vi "FPGA Main.vi"() -> ()   [LabVIEW 2016]
doc: "This FPGA Main VI contains a control loop running in parallel with an RT watchdog loop.\n- The Control Loop performs control calculations on four input channels in parallel, and outputs the results to four output channels.\n- The RT Watchdog Loop checks for a periodic 'pet' from the RT Main VI to ensure communications between RT and FPGA are maintained."
uses:
  <vilib>/LabVIEW Targets/FPGA/cRIO/shared/nicrio_ModuleControls/nicrio_cRIO-9239_DataRatesRing.ctl
  <vilib>/rvi/Emulation/niFpgaGetClockAttributes.vi
  <vilib>/rvi/Emulation/niFpgaSctlEmulationGetInTimedLoop.vi
  <vilib>/rvi/Emulation/niFpgaEmulationReportErrorSimple.vi
  <vilib>/rvi/Emulation/niFpgaProcessEmulError.vi
  <vilib>/rvi/eio/common/nirviEmuTemplatePropertySet_errors.vi
  <vilib>/rvi/eio/common/nirviEmuTemplateMethod_errors.vi
  <vilib>/rvi/interface/RandomDataEmulation/niFpgaRandomDataHandleErrors.vi
  <vilib>/rvi/Emulation/niFpgaCriticalErrorInLSC.vi
  <vilib>/eio/EIOPropertyNode/EIOPropertyNode.xnode
  <vilib>/eio/EIONode/EIONode.xnode
  <vilib>/rvi/DataTransferAndStorage/Container/XNode/niFpgaContainer.xnode
  <vilib>/rvi/interface/RandomDataEmulation/nirviRandomDataFpgaReadWriteTemplate.vi
  <vilib>/rvi/FXPMathLib/FxpMul/XNode/nifxpmath_Multiplier.xnode
  <vilib>/rvi/eio/common/nirviEmuTemplatePropertyGet_errors.vi
  <vilib>/rvi/eio/common/nirviEmuTemplatePropertyGet_noerrors.vi
  <vilib>/rvi/eio/common/nirviEmuTemplatePropertySet_noerrors.vi
  <vilib>/rvi/FXPMathLib/sim/FxpSim.dll
panel:
  in  "Stop":bool
  out "AI FIFO Full":bool
  out "AI AO Error":errorcluster
  out "AO FIFO Empty":bool
  in  "Loop Rate(uSec)":u32 caption="Loop Rate (uSec)"
  in  "Stop":bool
  in  "Amplitude":fxp<+/-,20,5>=10.0
  in  "Frequency (periods/tick)":fxp<+,32,0>=1.2499978765845299e-05
  in  "Data Rate":T1=1 items=["50.000 kS/s (NI 9239)"=1, "25.000 kS/s (NI 9239)"=2, "16.667 kS/s (NI 9239)"=3, "12.500 kS/s (NI 9239)"=4, "10.000 kS/s (NI 9239)"=5, "8.333 kS/s (NI 9239)"=6, "7.143 kS/s (NI 9239)"=7, "6.250 kS/s (NI 9239)"=8, "5.556 kS/s (NI 9239)"=9, "5.000 kS/s (NI 9239)"=10, "4.545 kS/s (NI 9239)"=11, "4.167 kS/s (NI 9239)"=12, "3.846 kS/s (NI 9239)"=13, "3.571 kS/s (NI 9239)"=14, "3.333 kS/s (NI 9239)"=15, "3.125 kS/s (NI 9239)"=16, "2.941 kS/s (NI 9239)"=17, "2.778 kS/s (NI 9239)"=18, "2.632 kS/s (NI 9239)"=19, "2.500 kS/s (NI 9239)"=20, "2.381 kS/s (NI 9239)"=21, "2.273 kS/s (NI 9239)"=22, "2.174 kS/s (NI 9239)"=23, "2.083 kS/s (NI 9239)"=24, "2.000 kS/s (NI 9239)"=25, "1.923 kS/s (NI 9239)"=26, "1.852 kS/s (NI 9239)"=27, "1.786 kS/s (NI 9239)"=28, "1.724 kS/s (NI 9239)"=29, "1.667 kS/s (NI 9239)"=30, "1.613 kS/s (NI 9239)"=31]
  out "FPGA Error":errorcluster
  out "Finished":bool
  in  "Stop":bool
  out "Module Underflow":bool
  out "DMA FIFO Full":bool
  out "Different Channel Count":bool
  out "Actual Loop Period (ticks)":u32
  out "First Read":bool
  in  "Number of Channels":i32=16
  in  "Channel Scale Array":fxp<+,24,12>[](array[numeric])=[0.0, 0.0, 0.0, 0.0, 0.0, 0.0, 0.0, 0.0, 0.0, 0.0, 0.0, 0.0, 0.0, 0.0, 0.0, 0.0]
  # "Essa VI é a interface direta entre o software (LabVIEW) e a FPGA.\nQualquer alteração mínima nela deve ser compilada, o que leva em torno de 20 minutos,  para poder ser executada."
  # "Reception Settings"
  # "Monitoring Values"
  # "Transmission"
  # "Supervision Analog"
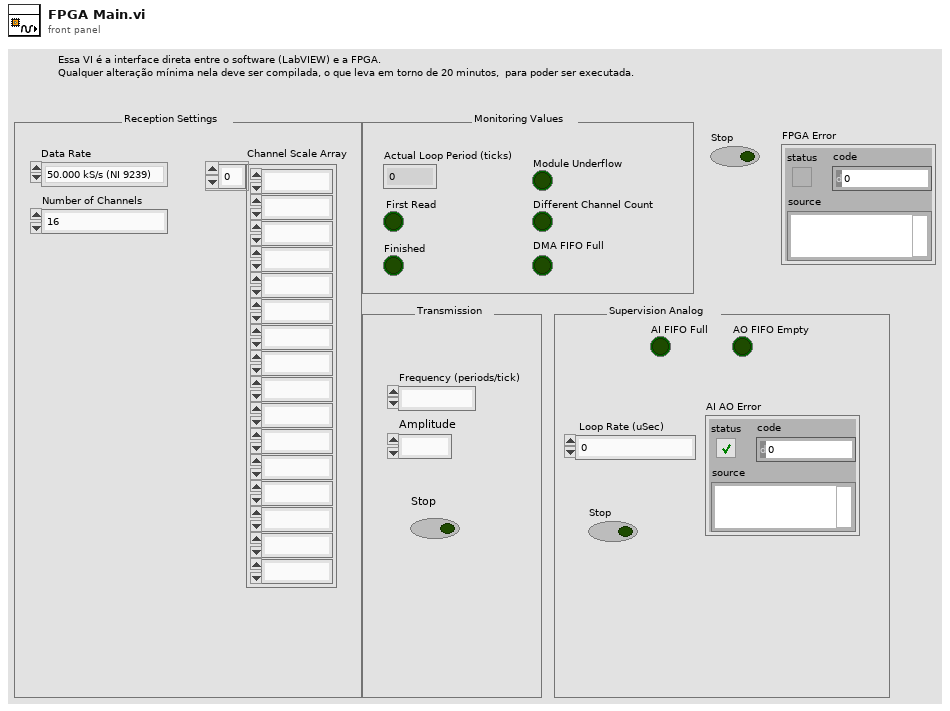
[diagram p1: front panel]
types:
  T1 = typedef "nicrio_cRIO-9239_DataRatesRing.ctl" = u8
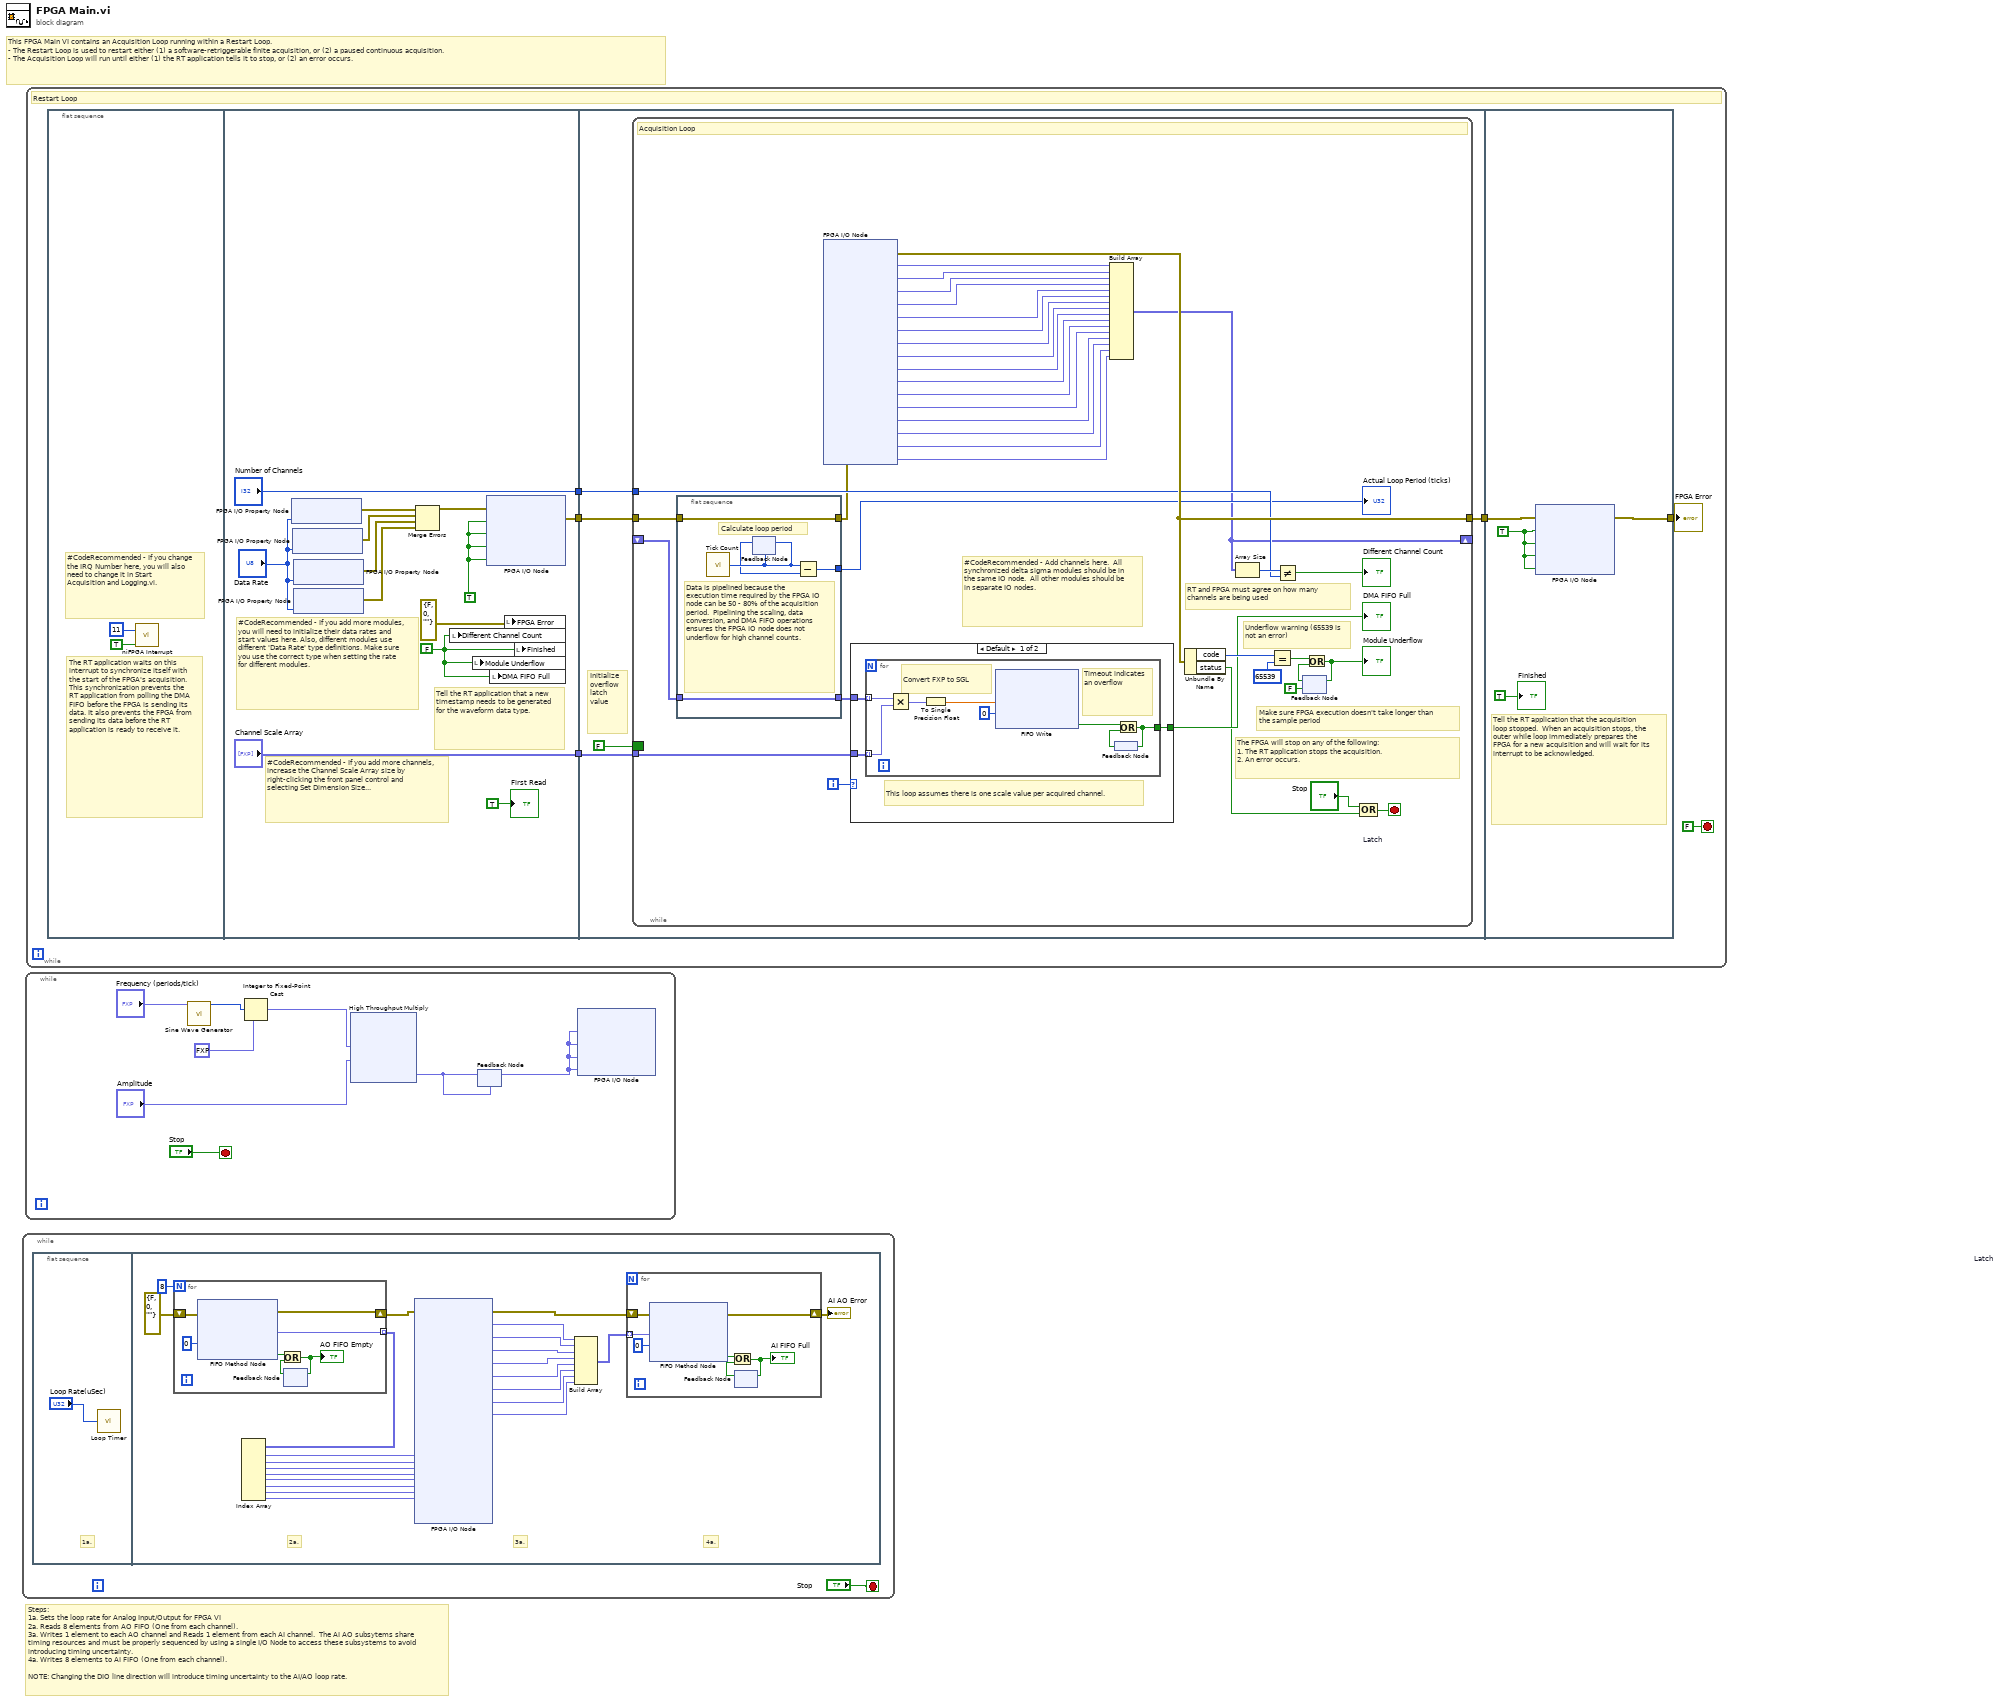
[diagram p0: block diagram]
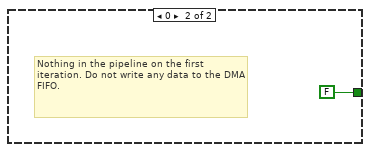
[diagram p2: hidden frame]
diagram:
  # "Steps:\n1a. Sets the loop rate for Analog Input/Output for FPGA VI\n2a. Reads 8 elements from AO FIFO (One from each channel).\n3a. Writes 1 element to each AO channel and Reads 1 element from each AI channel.  The AI AO subsytems share timing resources and must be properly sequenced by using a single I/O Node to access these subsystems to avoid introducing timing uncertainty.\n4a. Writes 8 elements to AI FIFO (One from each channel).\n\nNOTE: Changing the DIO line direction will introduce timing uncertainty to the AI/AO loop rate."
  # "This FPGA Main VI contains an Acquisition Loop running within a Restart Loop.\n- The Restart Loop is used to restart either (1) a software-retriggerable finite acquisition, or (2) a paused continuous acquisition.\n- The Acquisition Loop will run until either (1) the RT application tells it to stop, or (2) an error occurs."
  n1 = while {
    stop <- "Stop" stop-if-true
    n2 = flat-sequence {
      frame #0 {
        # "1a."
        n3 = call "Loop Timer"("Count(uSec)"="Loop Rate(uSec)") -> ()  [unwired: 1 out]
      }
      frame #1 {
        # "4a."
        # "3a."
        # "2a."
        n4 = for {
          N: 8 -> [_]
          tunnel: [w32] -> w14 mode=indexing
          shift-right: [w26] -> w3
          shift-left: errorcluster {"status"=FALSE, "code"=0, "source"=""} ("error out") -> [w27]
          n5 = xnode ("FIFO Method Node")("Timeout"=0, "error in (no error)"=w27) -> ("Element"=w32:fxp<+,16,3>, "Timed Out?"=w29:bool, "error out"=w26:errorcluster)  [unwired: 1 in, 1 out]
          n6 = feedback #1() -> (w30:bool)  [unwired: 1 in]
          n7 = Or(x=w29, y=w30) -> (x .or. y?=w31:bool)
          "AO FIFO Empty" <- w31
          n8 = feedback-in #1(w31) -> ()
        }
        n9 = Index Array(array=w14) -> (element #1=w13:fxp<+,16,3>, element #2=w9:fxp<+,16,3>, element #3=w10:fxp<+,16,3>, element #4=w11:fxp<+,16,3>, element #5=w12:fxp<+,16,3>, element #6=w8:fxp<+,16,3>, element #7=w7:fxp<+,16,3>, element #8=w6:fxp<+,16,3>)  [unwired: 8 in]
        n10 = xnode "FPGA I/O Node"("error in"=w3, "Mod2/AO0"=w13, "Mod2/AO1"=w9, "Mod2/AO2"=w10, "Mod2/AO3"=w11, "Mod2/AO4"=w12, "Mod2/AO5"=w8, "Mod2/AO6"=w7, "Mod2/AO7"=w6) -> ("error out"=w24:errorcluster, "Mod2/AI0"=w15:fxp<+,18,3>, "Mod2/AI1"=w16:fxp<+,18,3>, "Mod2/AI2"=w17:fxp<+,18,3>, "Mod2/AI3"=w18:fxp<+,18,3>, "Mod2/AI4"=w19:fxp<+,18,3>, "Mod2/AI5"=w20:fxp<+,18,3>, "Mod2/AI6"=w21:fxp<+,18,3>, "Mod2/AI7"=w22:fxp<+,18,3>)  [unwired: 16 in, 16 out]
        n11 = Build Array(w15, w16, w17, w18, w19, w20, w21, w22) -> (w23:fxp<+,18,3>[])
        n12 = for {
          tunnel: w23 -> [w39] mode=indexing
          shift-right: [w38] -> w25
          shift-left: w24 -> [w37]
          n13 = xnode ("FIFO Method Node")("Element"=w39, "Timeout"=0, "error in (no error)"=w37) -> ("Timed Out?"=w33:bool, "error out"=w38:errorcluster)  [unwired: 1 in, 1 out]
          n14 = feedback #2() -> (w35:bool)  [unwired: 1 in]
          n15 = Or(x=w33, y=w35) -> (x .or. y?=w34:bool)
          "AI FIFO Full" <- w34
          n16 = feedback-in #2(w34) -> ()
        }
        "AI AO Error" <- w25
      }
    }
  }
  n17 = while {
    stop <- "Stop" stop-if-true
    n18 = call "Sine Wave Generator"("frequency (periods/tick)"="Frequency (periods/tick)") -> ("sine out"=w46:i16)  [unwired: 14 in]
    n19 = Integer to Fixed-Point Cast(fixed-point type=fxp<+/-,16,1> 0.0, integer=w46) -> (fixed-point=w45:fxp<+/-,16,1>)
    n20 = xnode ("High Throughput Multiply")("x"=w45, "y"="Amplitude") -> ("x*y"=w42:fxp<+/-,20,5>)
    n21 = feedback-in #3(w42) -> ()
    n22 = feedback #3(w42) -> (w41:fxp<+/-,20,5>)
    n23 = xnode "FPGA I/O Node"("Mod1/AO0"=w41, "Mod1/AO1"=w41, "Mod1/AO2"=w41, "Mod1/AO3"=w41) -> ()  [unwired: 4 in, 4 out]
  }
  n24 = while {
    stop <- FALSE stop-if-true
    # "Restart Loop"
    n25 = flat-sequence {
      tunnel: [w68] -> w52
      tunnel: ["Channel Scale Array"] -> w51
      tunnel: ["Number of Channels"] -> w50
      tunnel: w52 -> [w72]
      tunnel: w51 -> [w71]
      tunnel: w50 -> [w73]
      tunnel: [w70] -> w49
      tunnel: w49 -> [w131]
      tunnel: [w130] -> w48
      frame #0 {
        # "#CodeRecommended - If you change the IRQ Number here, you will also need to change it in Start Acquisition and Logging.vi."
        # "The RT application waits on this interrupt to synchronize itself with the start of the FPGA's acquisition.  This synchronization prevents the RT application from polling the DMA FIFO before the FPGA is sending its data. It also prevents the FPGA from sending its data before the RT application is ready to receive it."
        n26 = call <vilib>:"niFPGA Interrupt.vi"("Wait Until Cleared (F)"=TRUE ("Wait Until Cleared"), "IRQ Number (0)"=u8 11 ("IRQ Number")) -> ()  [unwired: 1 in]
      }
      frame #1 {
        w66 = FALSE ("Module Underflow")
        w61 = TRUE ("Mod1/Start")
        # "Tell the RT application that a new timestamp needs to be generated for the waveform data type."
        # "#CodeRecommended - If you add more channels, increase the Channel Scale Array size by right-clicking the front panel control and selecting Set Dimension Size..."
        # "#CodeRecommended - If you add more modules, you will need to initialize their data rates and start values here. Also, different modules use different 'Data Rate' type definitions. Make sure you use the correct type when setting the rate for different modules."
        n27 = xnode "FPGA I/O Property Node"("Data Rate"="Data Rate") -> ("error out"=w59:errorcluster)  [unwired: 2 in, 1 out]
        n28 = xnode "FPGA I/O Property Node"("Data Rate"="Data Rate") -> ("error out"=w60:errorcluster)  [unwired: 2 in, 1 out]
        n29 = xnode "FPGA I/O Property Node"("Data Rate"="Data Rate") -> ("error out"=w58:errorcluster)  [unwired: 2 in, 1 out]
        n30 = xnode "FPGA I/O Property Node"("Data Rate"="Data Rate") -> ("error out"=w57:errorcluster)  [unwired: 2 in, 1 out]
        n31 = Merge Errors(w59, w60, w58, w57) -> (w56:errorcluster)
        n32 = local write "Different Channel Count"(w66) -> ()
        n33 = local write "Module Underflow"(w66) -> ()
        n34 = xnode "FPGA I/O Node"("error in"=w56, "Mod3/Start"=w61, "Mod4/Start"=w61, "Mod5/Start"=w61, "Mod6/Start"=w61) -> ("error out"=w68:errorcluster)  [unwired: 4 in, 4 out]
        n35 = local write "DMA FIFO Full"(w66) -> ()
        n36 = local write "FPGA Error"(errorcluster {"status"=FALSE, "code"=0, "source"=""} ("FPGA Error")) -> ()
        n37 = local write "Finished"(w66) -> ()
        "First Read" <- TRUE ("First Read")
      }
      frame #2 {
        # "Initialize overflow latch value"
        n38 = while {
          tunnel: w72 -> [w103]
          tunnel: [w108] -> w70
          shift-right: [w93] -> _
          shift-left: _ -> [w95]
          tunnel: w73 -> [w105]
          tunnel: w71 -> [w97]
          border: FALSE ("Overflow\nLatch") -> [_]
          i -> [w86]
          stop <- w111 stop-if-true
          # "Underflow warning (65539 is not an error)"
          # "The FPGA will stop on any of the following:\n1. The RT application stops the acquisition.\n2. An error occurs."
          # "#CodeRecommended - Add channels here.  All synchronized delta sigma modules should be in the same IO node.  All other modules should be in separate IO nodes."
          # "RT and FPGA must agree on how many channels are being used"
          # "Make sure FPGA execution doesn't take longer than the sample period"
          # "Acquisition Loop"
          n39 = flat-sequence {
            tunnel: [w128] -> w102
            tunnel: w103 -> [w128]
            tunnel: [w125] -> w101
            tunnel: w95 -> [w124]
            tunnel: [w124] -> w96
            frame #0 {
              # "Data is pipelined because the execution time required by the FPGA IO node can be 50 - 80% of the acquisition period.  Pipelining the scaling, data conversion, and DMA FIFO operations ensures the FPGA IO node does not underflow for high channel counts."
              # "Calculate loop period"
              n40 = call "Tick Count"() -> ("Tick Count(Ticks)"=w127:u32)
              n41 = feedback-in #4(w127) -> ()
              n42 = feedback #4(w127) -> (w126:u32)
              n43 = Subtract(x=w127, y=w126) -> (x-y=w125:u32)
            }
          }
          n44 = xnode "FPGA I/O Node"("error in"=w102) -> ("error out"=w108:errorcluster, "Mod3/AI0"=w100:fxp<+/-,24,5>, "Mod3/AI1"=w94:fxp<+/-,24,5>, "Mod3/AI2"=w99:fxp<+/-,24,5>, "Mod3/AI3"=w98:fxp<+/-,24,5>, "Mod4/AI0"=w74:fxp<+/-,24,5>, "Mod4/AI1"=w75:fxp<+/-,24,5>, "Mod4/AI2"=w76:fxp<+/-,24,5>, "Mod4/AI3"=w77:fxp<+/-,24,5>, "Mod5/AI0"=w78:fxp<+/-,24,5>, "Mod5/AI1"=w79:fxp<+/-,24,5>, "Mod5/AI2"=w80:fxp<+/-,24,5>, "Mod5/AI3"=w81:fxp<+/-,24,5>, "Mod6/AI0"=w82:fxp<+/-,24,5>, "Mod6/AI1"=w83:fxp<+/-,24,5>, "Mod6/AI2"=w84:fxp<+/-,24,5>, "Mod6/AI3"=w85:fxp<+/-,24,5>)  [unwired: 16 in, 16 out]
          n45 = case shown="Default" w86 {
            tunnel: [w114 FALSE] -> w107
            tunnel: w97 -> [w113 _]
            tunnel: w96 -> [w112 _]
            frame Default {
              # "This loop assumes there is one scale value per acquired channel."
              n46 = for {
                tunnel: [w120] -> w114
                tunnel: w112 -> [w118] mode=indexing
                tunnel: w113 -> [w117] mode=indexing
                # "Timeout indicates an overflow"
                # "Convert FXP to SGL"
                n47 = Multiply(x=w118, y=w117) -> (x*y=w116:fxp<+/-,48,17>)
                n48 = To Single Precision Float(number=w116) -> (single precision float=w115:sgl)
                n49 = xnode ("FIFO Write")("Element"=w115, "Timeout"=0) -> ("Timed Out?"=w122:bool)  [unwired: 1 in, 1 out]
                n50 = feedback #5 "Latch"() -> (w121:bool)
                n51 = Or(x=w122, y=w121) -> (x .or. y?=w120:bool)
                n52 = feedback-in #5(w120) -> ()
              }
            }
            frame 0 {
              # "Nothing in the pipeline on the first iteration. Do not write any data to the DMA FIFO."
            }
          }
          "DMA FIFO Full" <- w107
          n53 = Build Array(w100, w94, w99, w98, w74, w75, w76, w77, w78, w79, w80, w81, w82, w83, w84, w85) -> (w93:fxp<+/-,24,5>[])
          n54 = Unbundle By Name(w108) -> ("code"=w109:i32, "status"=w88:bool)
          n55 = Array Size(array=w93) -> (size(s)=w106:i32)
          n56 = Equal?(x=w109, y=65539) -> (x = y?=w90:bool)
          n57 = Not Equal?(x=w106, y=w105) -> (x != y?=→"Different Channel Count":bool)
          n58 = feedback #6 "Latch"(FALSE) -> (w92:bool)
          n59 = Or(x=w90, y=w92) -> (x .or. y?=w89:bool)
          "Module Underflow" <- w89
          n60 = feedback-in #6(w89) -> ()
          n61 = Compound Arithmetic op=OR("Stop", w88) -> (w111:bool)
          "Actual Loop Period (ticks)" <- w101
        }
      }
      frame #3 {
        w129 = TRUE ("Mod1/Stop")
        # "Tell the RT application that the acquisition loop stopped.  When an acquisition stops, the outer while loop immediately prepares the FPGA for a new acquisition and will wait for its interrupt to be acknowledged."
        n62 = xnode "FPGA I/O Node"("error in"=w131, "Mod3/Stop"=w129, "Mod4/Stop"=w129, "Mod5/Stop"=w129, "Mod6/Stop"=w129) -> ("error out"=w130:errorcluster)  [unwired: 4 in, 4 out]
        "Finished" <- TRUE ("Finished")
      }
    }
    "FPGA Error" <- w48
  }
